vi "Octal Channel Engine.vi"(0 "Notifier Name":string, 11 "AOTF Index":string[](array[string])) -> ()   [LabVIEW 2016]
uses:
  Octal Channel Type Defs/Octal Channel AOTF Config.ctl
  AOTF Controls/AOTF Notifier Element.ctl
  AOTF Controls/AOTF Actions.ctl
  Program Files/Crystal Technology/Developer/AotfLibrary/Dll/AotfLibrary.dll
panel:
  in  "Wavelength (nm)":u16(ring) items=["642", "560", "542"]
  in  "Line On/Off":bool
  out "Controller Response":string
  in  "Blank All":bool=TRUE
  in  "Quit":bool
  in  "Power (%)":dbl
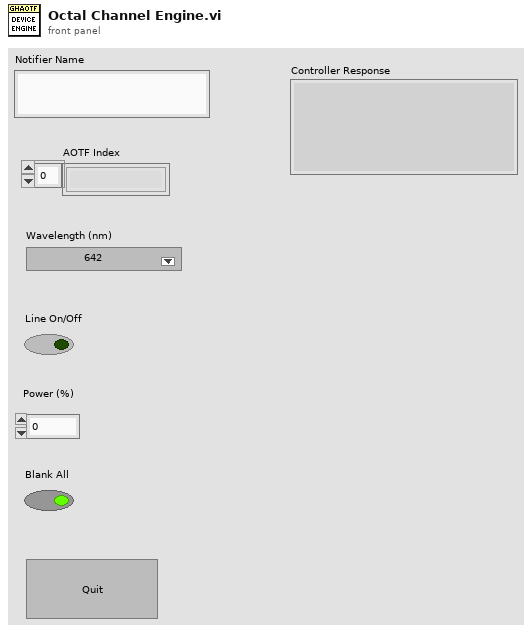
[diagram p1: front panel]
types:
  T1 = typedef "AOTF Notifier Element.ctl" = cluster{"AOTF Action":T2, "Laser Line":string, "Power (%)":dbl, "Beam Blank On/Off":bool, "Line On/Off":bool, "Error":errorcluster, "Wavelengths (nm)":string[]}
  T2 = typedef "AOTF Actions.ctl" = enum16{"Error Check", "Blank", "Line On/Off", "Set Power", "Status", "Quit"}
  T3 = typedef "Octal Channel AOTF Config.ctl" = cluster{"Wavelength (nm)":u16[], "Channel Number":u8[], "Frequency (MHz)":dbl[], "Max Power":dbl[]}
  T4 = enum32{"Invalid", "Standard", "Closed", "Hidden", "Minimized", "Maximized"}
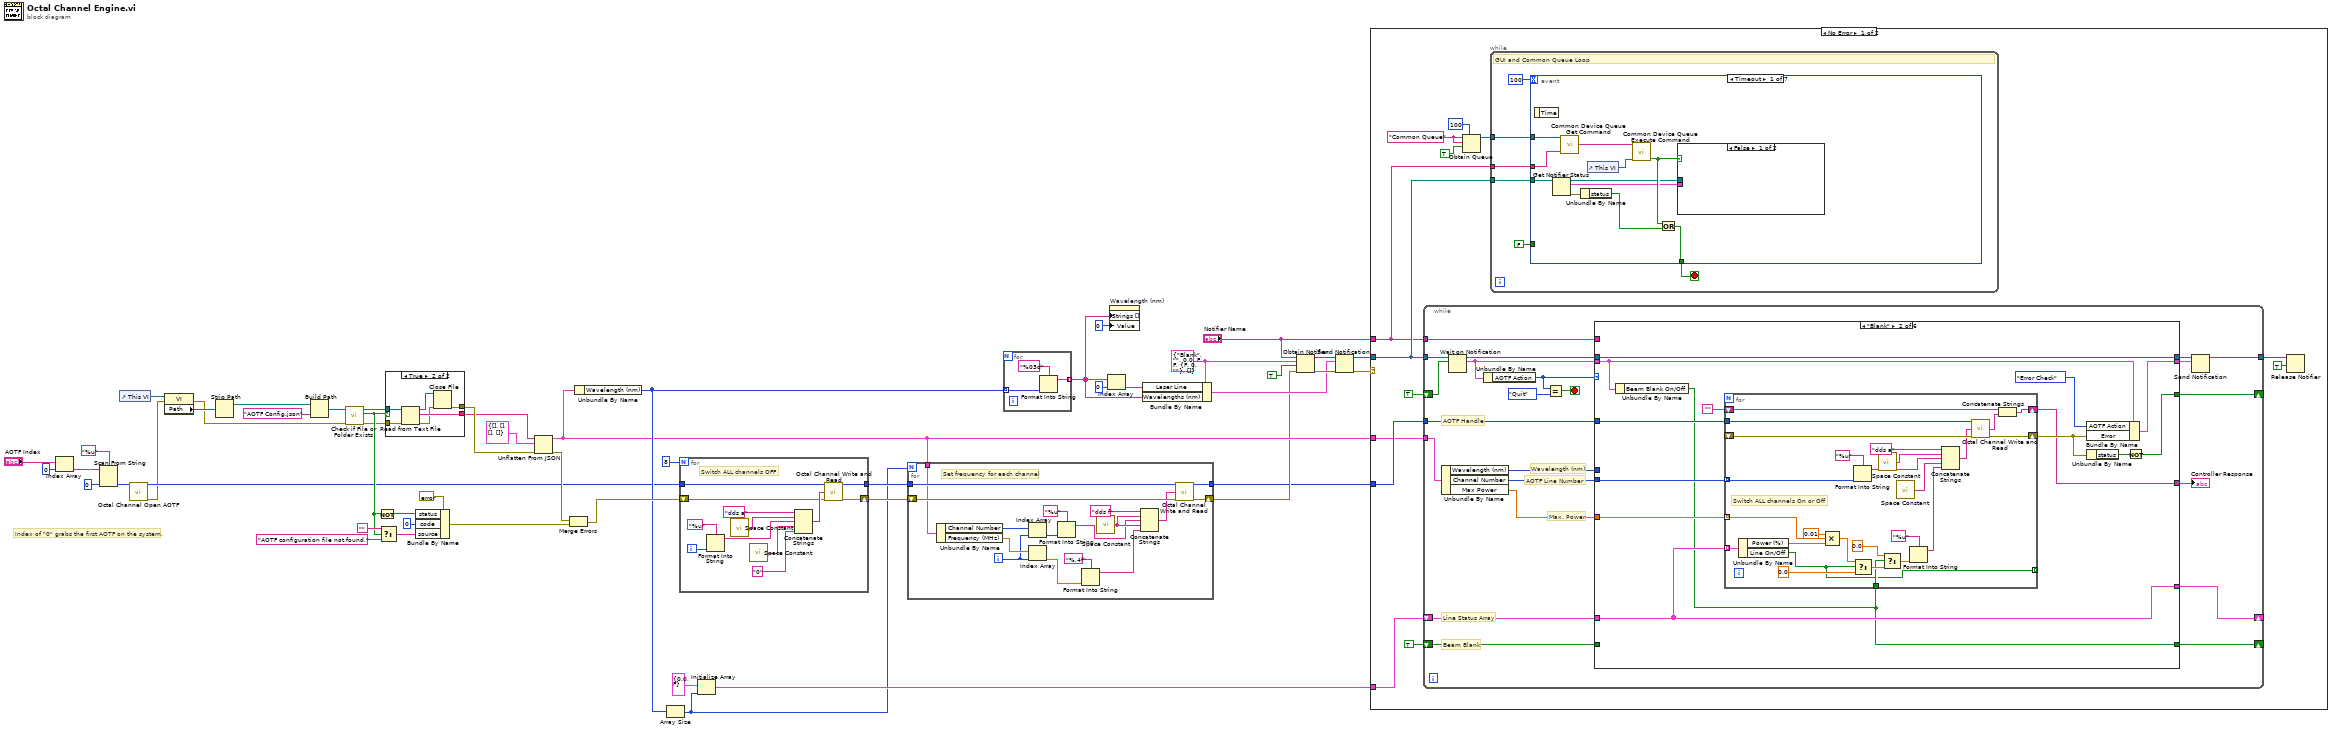
[diagram p0: block diagram]
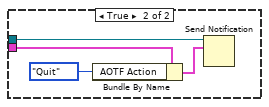
[diagram p2: hidden frame]
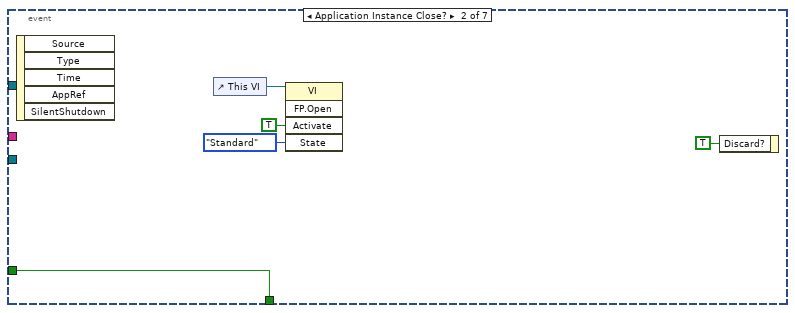
[diagram p3: hidden frame]
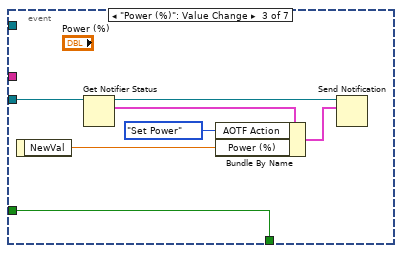
[diagram p4: hidden frame]
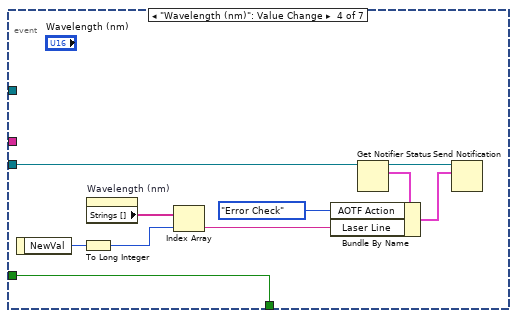
[diagram p5: hidden frame]
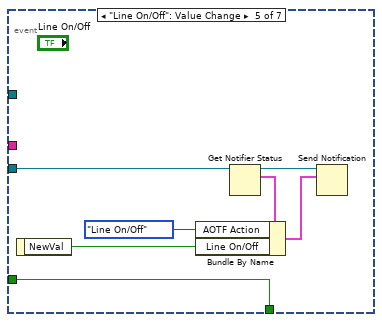
[diagram p6: hidden frame]
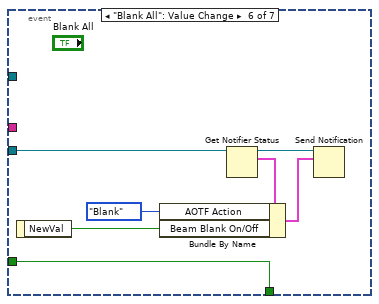
[diagram p7: hidden frame]
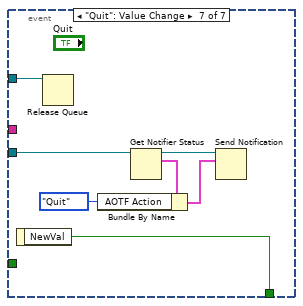
[diagram p8: hidden frame]
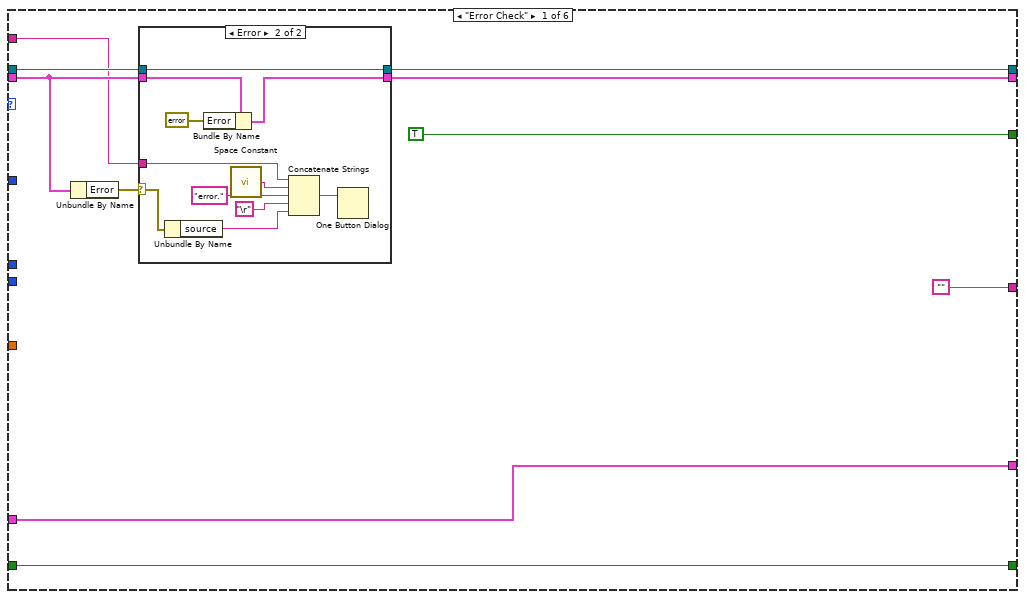
[diagram p9: hidden frame]
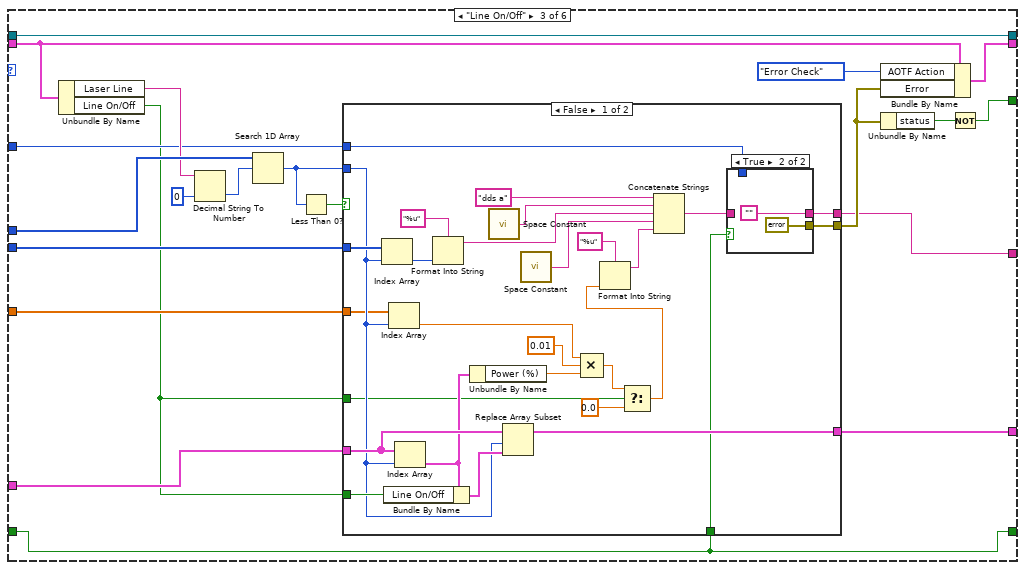
[diagram p11: hidden frame]
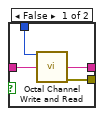
[diagram p12: hidden frame]
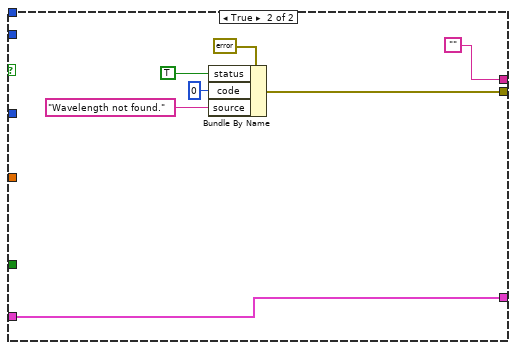
[diagram p13: hidden frame]
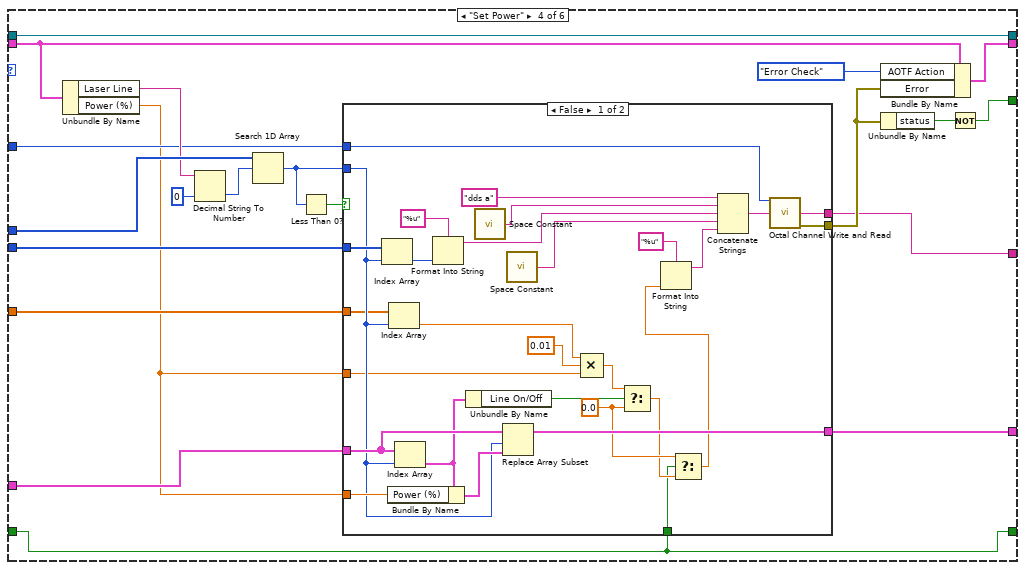
[diagram p14: hidden frame]
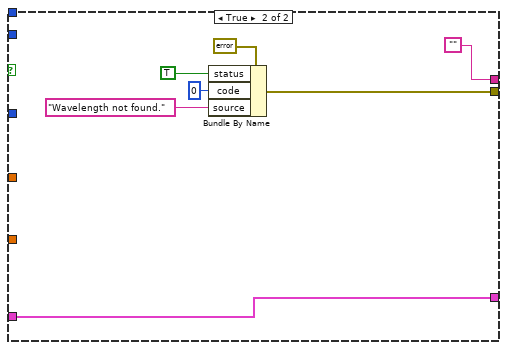
[diagram p15: hidden frame]
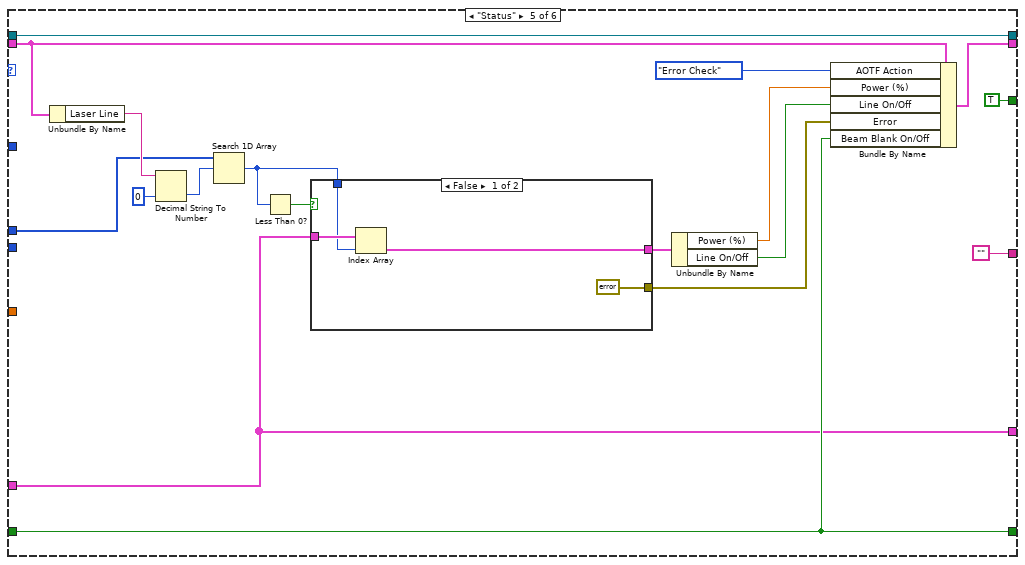
[diagram p16: hidden frame]
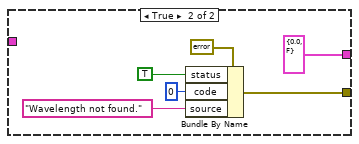
[diagram p17: hidden frame]
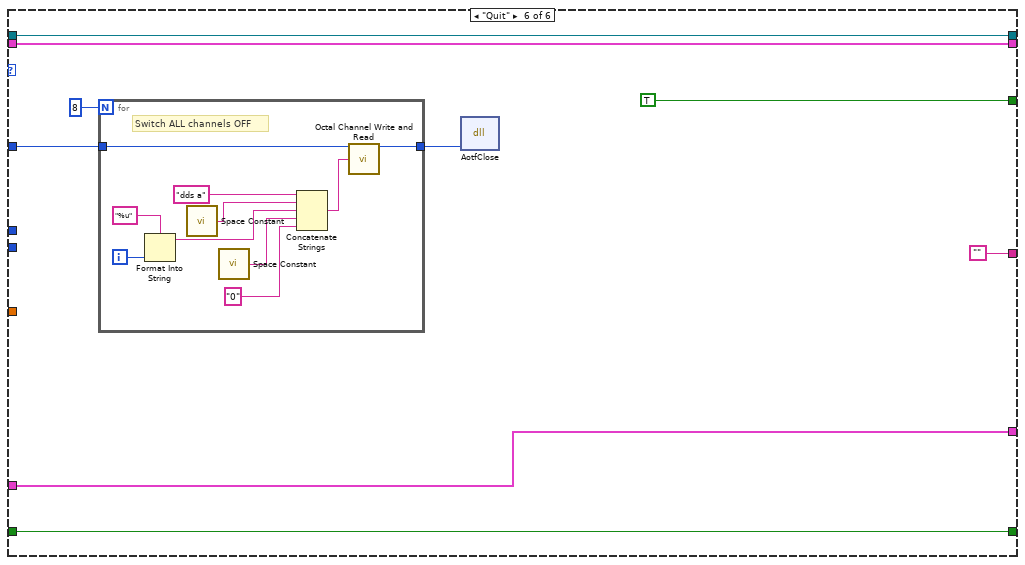
[diagram p18: hidden frame]
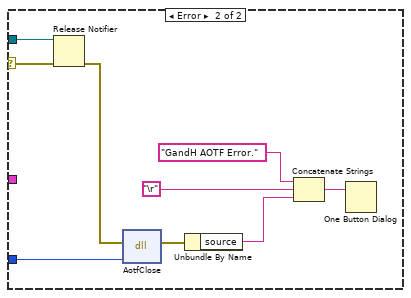
[diagram p19: hidden frame]
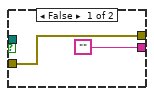
[diagram p20: hidden frame]
diagram:
  w17 = T1 {"AOTF Action"=enum."Blank", "Laser Line"="", "Power (%)"=0.0, "Beam Blank On/Off"=FALSE, "Line On/Off"=FALSE, "Error"={"status"=FALSE, "code"=0, "source"=""}, "Wavelengths (nm)"=[]} ("AOTFQueueCtrl")
  # "Index of \"0\" grabs the first AOTF on the system."
  n1 = Index Array(array="AOTF Index", index=0) -> (element=w4:string)
  n2 = Scan From String(format string="%u", input string=w4, default 1=0 ("AOTF Index")) -> (output 1=w1:i32)  [unwired: 2 in, 3 out]
  n3 = control-ref of="This VI"() -> (w51:refnum<vi>)
  n4 = call "Octal Channel Open AOTF.vi"("AOTF Index"=w1) -> ("AOTF Handle"=w15:u64, "Error Out"=w14:errorcluster)  [unwired: 13 in]
  n5 = property class="VI"(reference=w51, error in=w14) -> (error out=w38:errorcluster, "Path"=w50:path)  [unwired: 1 out]
  n6 = Strip Path(path=w50) -> (stripped path=w49:path)  [unwired: 1 out]
  n7 = Build Path(base path=w49, name or relative path="AOTF Config.json") -> (appended path=w47:path)
  n8 = call <vilib>:"Check if File or Folder Exists.vi"("error in (no error)"=w38, "path"=w47) -> ("error out"=w37:errorcluster, "file or folder exists?"=w40:bool, "dup path"=w39:path)  [unwired: 7 in]
  n9 = Not(x=w40) -> (.not. x?=w45:bool)
  n10 = Select(t="", s=w40, f="AOTF configuration file not found." ("source")) -> (s? t:f=w41:string)
  n11 = case shown="True" w40 {
    tunnel: w39 -> [_ w59]
    tunnel: ["" w58] -> w33
    tunnel: w37 -> [w52 w56]
    tunnel: [w52 w54] -> w36
    frame False {
    }
    frame True {
      n12 = Read from Text File(file (use dialog)=w59, error in=w56) -> (refnum out=w57:refnum<file>, text=w58:string, error out=w55:errorcluster)  [unwired: 2 in, 1 out]
      n13 = Close File(refnum=w57, error in=w55) -> (error out=w54:errorcluster)  [unwired: 1 out]
    }
  }
  n14 = Bundle By Name(cluster=errorcluster {"status"=FALSE, "code"=0, "source"=""} ("Error"), "status"=w45, "code"=0, "source"=w41) -> (w34:errorcluster)
  n15 = Unflatten From JSON(JSON string=w33, type and defaults=T3 {"Wavelength (nm)"=[], "Channel Number"=[], "Frequency (MHz)"=[], "Max Power"=[]} ("AOTF Config"), error in (no error)=w36) -> (value=w9:T3, error out=w35:errorcluster)  [unwired: 4 in]
  n16 = Merge Errors(w35, w34) -> (w29:errorcluster)
  n17 = Unbundle By Name(w9) -> ("Wavelength (nm)"=w28:u16[])
  n18 = Array Size(array=w28) -> (size(s)=w10:i32)
  n19 = for {
    N: 8 -> [_]
    shift-right: [w63] -> w12
    shift-left: w29 -> [w62]
    tunnel: w15 -> [w61]
    tunnel: [w60] -> w11
    i -> [w64]
    # "Switch ALL channels OFF"
    n20 = Format Into String(format string="%u", w64) -> (resulting string=w71:string)  [unwired: 2 in, 1 out]
    n21 = call <vilib>:"Space Constant.vi"() -> ("String"=w66:string)
    n22 = call <vilib>:"Space Constant.vi"() -> ("String"=w67:string)
    n23 = Concatenate Strings("dds a", w66, w71, w67, "0") -> (w69:string)
    n24 = call "Octal Channel Write and Read.vi"("hAotfController"=w61, "Command"=w69, "Error In"=w62) -> ("hAotfController (Dup)"=w60:u64, "Error Out"=w63:errorcluster)  [unwired: 10 in, 1 out]
  }
  n25 = Initialize Array(cluster{"Power (%)":dbl, "Line On/Off":bool} {"Power (%)"=0.0, "Line On/Off"=FALSE} ("Line Staus Cluster"), w10) -> (w30:cluster{"Power (%)":dbl, "Line On/Off":bool}[])
  n26 = for {
    N: w10 -> [_]
    shift-right: [w80] -> w8
    shift-left: w12 -> [w87]
    tunnel: w11 -> [w88]
    tunnel: w9 -> [w86]
    tunnel: [w72] -> w7
    i -> [w83]
    # "Set frequency for each channel"
    n27 = Unbundle By Name(w86) -> ("Channel Number"=w85:u8[], "Frequency (MHz)"=w84:dbl[])
    n28 = Index Array(array=w85, index=w83) -> (element=w77:u8)
    n29 = Index Array(array=w84, index=w83) -> (element=w74:dbl)
    n30 = Format Into String(format string="%u", w77) -> (resulting string=w76:string)  [unwired: 2 in, 1 out]
    n31 = Format Into String(format string="%.4f", w74) -> (resulting string=w73:string)  [unwired: 2 in, 1 out]
    n32 = call <vilib>:"Space Constant.vi"() -> ("String"=w81:string)
    n33 = Concatenate Strings("dds f", w81, w76, w81, w73) -> (w79:string)
    n34 = call "Octal Channel Write and Read.vi"("hAotfController"=w88, "Command"=w79, "Error In"=w87) -> ("hAotfController (Dup)"=w72:u64, "Error Out"=w80:errorcluster)  [unwired: 10 in, 1 out]
  }
  n35 = for {
    tunnel: w28 -> [w91] mode=indexing
    tunnel: [w90] -> w27 mode=indexing
    n36 = Format Into String(format string="%03d", w91) -> (resulting string=w90:string)  [unwired: 2 in, 1 out]
  }
  n37 = Index Array(array=w27, index=0) -> (element=w25:string)
  n38 = property on="Wavelength (nm)" class="Ring (strict)"("Strings []"=w27, "Value"=u16 0 ("index")) -> ()  [unwired: 2 in, 2 out]
  n39 = Bundle By Name(cluster=w17, "Laser Line"=w25, "Wavelengths (nm)"=w27) -> (w16:T1)
  n40 = Obtain Notifier(name (unnamed)="Notifier Name", notification data type=w17, create if not found? (T)=TRUE, error in (no error)=w8) -> (notifier out=w21:refnum<notifier>, error out=w20:errorcluster)  [unwired: 1 out]
  n41 = Send Notification(notification=w16, notifier=w21, error in (no error)=w20) -> (notifier out=w19:refnum<notifier>, error out=w18:errorcluster)
  n42 = case shown="No Error" w18 {
    selector: w18 -> [_ w427]
    tunnel: w19 -> [w100 w428]
    tunnel: "Notifier Name" -> [w96 _]
    tunnel: w7 -> [w95 w420]
    tunnel: w30 -> [w94 _]
    tunnel: w9 -> [w92 _]
    frame No Error {
      w104 = "Common Queue" ("Unique Notifier Name")
      n43 = while {
        tunnel: w100 -> [w190]
        shift-right: [w181] -> _
        shift-left: TRUE ("ignore previous (F)") -> [w189]
        tunnel: [w180] -> w98
        tunnel: w96 -> [w179]
        tunnel: w95 -> [w178]
        shift-right: [w173] -> _
        shift-left: w94 -> [w176]
        shift-right: [w174] -> _
        shift-left: TRUE -> [w175]
        tunnel: w92 -> [w172]
        stop <- w184 stop-if-true
        # "Wavelength (nm)"
        # "AOTF Line Number"
        # "Line Status Array"
        # "Beam Blank"
        # "AOTF Handle"
        # "Max. Power"
        n44 = Unbundle By Name(w172) -> ("Wavelength (nm)"=w171:u16[], "Channel Number"=w170:u8[], "Max Power"=w169:dbl[])
        n45 = Wait on Notification(notifier=w190, ignore previous (F)=w189) -> (notifier out=w188:refnum<notifier>, notification=w187:T1)  [unwired: 2 in, 2 out]
        n46 = Unbundle By Name(w187) -> ("AOTF Action"=w186:T2)
        n47 = Equal?(x=w186, y=AOTF_Actions."Quit") -> (x = y?=w184:bool)
        n48 = case shown="\"Blank\"" w186 {
          tunnel: w188 -> [w200 w227 w270 w332 w389 w409]
          tunnel: w187 -> [w198 w226 w272 w334 w384 w408]
          tunnel: [w196 w227 w270 w332 w389 w409] -> w183
          tunnel: [w195 w225 w271 w333 w380 w408] -> w182
          tunnel: [TRUE w222 w262 w324 TRUE TRUE] -> w181
          tunnel: w179 -> [w197 _ _ _ _ _]
          tunnel: w171 -> [_ _ w267 w329 w385 _]
          tunnel: w170 -> [_ w220 w264 w326 _ _]
          tunnel: w169 -> [_ w218 w257 w319 _ _]
          tunnel: w178 -> [_ w221 w258 w320 _ w402]
          tunnel: ["" w214 w255 w317 "" ""] -> w177
          tunnel: w176 -> [w192 w217 w261 w323 w373 w405]
          tunnel: w175 -> [w191 _ w254 w316 w374 w404]
          tunnel: [w191 w215 w254 w316 w374 w404] -> w174
          tunnel: [w192 w217 w260 w322 w373 w405] -> w173
          frame "Error Check" {
            n49 = Unbundle By Name(w198) -> ("Error"=w199:errorcluster)
            n50 = case shown="Error" w199 {
              selector: w199 -> [_ w206]
              tunnel: w198 -> [w201 w210]
              tunnel: [w202 w208] -> w196
              tunnel: w200 -> [w202 w208]
              tunnel: w197 -> [_ w205]
              tunnel: [w201 w207] -> w195
              frame No Error {
              }
              frame Error {
                n51 = Unbundle By Name(w206) -> ("source"=w204:string)
                n52 = Bundle By Name(cluster=w210, "Error"=errorcluster {"status"=FALSE, "code"=0, "source"=""}) -> (w207:T1)
                n53 = call <vilib>:"Space Constant.vi"() -> ("String"=w213:string)
                n54 = Concatenate Strings(w205, w213, "error." ("string"), "\r", w204) -> (w211:string)
                n55 = One Button Dialog(message=w211) -> ()  [unwired: 1 in, 1 out]
              }
            }
          }
          frame "Blank" {
            n56 = Unbundle By Name(w226) -> ("Beam Blank On/Off"=w215:bool)
            n57 = for {
              shift-right: [w248] -> w219
              shift-left: _ -> [w247]
              tunnel: w221 -> [w246]
              tunnel: w217 -> [w244] mode=indexing
              tunnel: w220 -> [w245] mode=indexing
              tunnel: w218 -> [w242] mode=indexing
              tunnel: w215 -> [w238]
              shift-right: [w233] -> w214
              shift-left: "" -> [w234]
              tunnel: [w229] -> _ mode=indexing
              # "Switch ALL channels On or Off"
              n58 = Unbundle By Name(w244) -> ("Power (%)"=w228:dbl, "Line On/Off"=w229:bool)
              n59 = Compound Arithmetic op=MULTIPLY(0.01 ("value"), w242, w228) -> (w241:dbl)
              n60 = Format Into String(format string="%u", w245) -> (resulting string=w253:string)  [unwired: 2 in, 1 out]
              n61 = Select(t=w241, s=w229, f=0.0) -> (s? t:f=w239:dbl)
              n62 = call <vilib>:"Space Constant.vi"() -> ("String"=w250:string)
              n63 = Select(t=0.0, s=w238, f=w239) -> (s? t:f=w236:dbl)
              n64 = call <vilib>:"Space Constant.vi"() -> ("String"=w251:string)
              n65 = Format Into String(format string="%u", w236) -> (resulting string=w235:string)  [unwired: 2 in, 1 out]
              n66 = Concatenate Strings("dds a", w250, w253, w251, w235) -> (w230:string)
              n67 = call "Octal Channel Write and Read.vi"("hAotfController"=w246, "Command"=w230, "Error In"=w247) -> ("Response"=w232:string, "Error Out"=w248:errorcluster)  [unwired: 10 in, 1 out]
              n68 = Concatenate Strings(w234, w232) -> (w233:string)
            }
            n69 = Bundle By Name(cluster=w226, "AOTF Action"=AOTF_Actions."Error Check", "Error"=w219) -> (w225:T1)
            n70 = Unbundle By Name(w219) -> ("status"=w223:bool)
            n71 = Not(x=w223) -> (.not. x?=w222:bool)
          }
          frame "Line On/Off" {
            n72 = Unbundle By Name(w272) -> ("Laser Line"=w266:string, "Line On/Off"=w256:bool)
            n73 = Decimal String To Number(string=w266, default (0L)=u16 0 ("default (0 I32)")) -> (number=w269:u16)  [unwired: 1 in, 1 out]
            n74 = Search 1D Array(1D array=w267, element=w269) -> (index of element=w259:i32)  [unwired: 1 in]
            n75 = Less Than 0?(x=w259) -> (x < 0?=w265:bool)
            n76 = case shown="False" w265 {
              tunnel: w264 -> [w302 _]
              tunnel: [w297 w311] -> w263
              tunnel: [w278 ""] -> w255
              tunnel: w261 -> [w301 w309]
              tunnel: [w300 w309] -> w260
              tunnel: w256 -> [w298 _]
              tunnel: w259 -> [w288 _]
              tunnel: w258 -> [w289 _]
              tunnel: w257 -> [w287 _]
              tunnel: w256 -> [w281 _]
              tunnel: w254 -> [w275 _]
              frame False {
                n77 = Index Array(array=w302, index=w288) -> (element=w291:u8)
                n78 = Index Array(array=w287, index=w288) -> (element=w282:dbl)
                n79 = Index Array(array=w301, index=w288) -> (element=w285:cluster{"Power (%)":dbl, "Line On/Off":bool})
                n80 = Bundle By Name(cluster=w285, "Line On/Off"=w298) -> (w299:cluster{"Power (%)":dbl, "Line On/Off":bool})
                n81 = Format Into String(format string="%u", w291) -> (resulting string=w292:string)  [unwired: 2 in, 1 out]
                n82 = Unbundle By Name(w285) -> ("Power (%)"=w284:dbl)
                n83 = call <vilib>:"Space Constant.vi"() -> ("String"=w295:string)
                n84 = Replace Array Subset(array=w301, new element=w299, index=w288) -> (w300:cluster{"Power (%)":dbl, "Line On/Off":bool}[])
                n85 = call <vilib>:"Space Constant.vi"() -> ("String"=w294:string)
                n86 = Compound Arithmetic op=MULTIPLY(w282, 0.01 ("value"), w284) -> (w286:dbl)
                n87 = Select(t=w286, s=w281, f=0.0) -> (s? t:f=w276:dbl)
                n88 = Format Into String(format string="%u", w276) -> (resulting string=w279:string)  [unwired: 2 in, 1 out]
                n89 = Concatenate Strings("dds a", w295, w292, w294, w279) -> (w290:string)
                n90 = case shown="True" w275 {
                  tunnel: [w306 errorcluster {"status"=FALSE, "code"=0, "source"=""} ("Error Out")] -> w297
                  tunnel: w290 -> [w305 _]
                  tunnel: w289 -> [w304 _]
                  tunnel: [w303 ""] -> w278
                  frame False {
                    n91 = call "Octal Channel Write and Read.vi"("hAotfController"=w304, "Command"=w305) -> ("Response"=w303:string, "Error Out"=w306:errorcluster)  [unwired: 11 in, 1 out]
                  }
                  frame True {
                  }
                }
              }
              frame True {
                n92 = Bundle By Name(cluster=errorcluster {"status"=FALSE, "code"=0, "source"=""} ("error out"), "status"=TRUE, "code"=0, "source"="Wavelength not found.") -> (w311:errorcluster)
              }
            }
            n93 = Bundle By Name(cluster=w272, "AOTF Action"=AOTF_Actions."Error Check", "Error"=w263) -> (w271:T1)
            n94 = Unbundle By Name(w263) -> ("status"=w273:bool)
            n95 = Not(x=w273) -> (.not. x?=w262:bool)
          }
          frame "Set Power" {
            n96 = Unbundle By Name(w334) -> ("Laser Line"=w328:string, "Power (%)"=w318:dbl)
            n97 = Decimal String To Number(string=w328, default (0L)=u16 0 ("default (0 I32)")) -> (number=w331:u16)  [unwired: 1 in, 1 out]
            n98 = Search 1D Array(1D array=w329, element=w331) -> (index of element=w321:i32)  [unwired: 1 in]
            n99 = Less Than 0?(x=w321) -> (x < 0?=w327:bool)
            n100 = case shown="False" w327 {
              tunnel: w326 -> [w365 _]
              tunnel: [w360 w368] -> w325
              tunnel: [w343 ""] -> w317
              tunnel: w323 -> [w364 w366]
              tunnel: [w363 w366] -> w322
              tunnel: w318 -> [w361 _]
              tunnel: w321 -> [w351 _]
              tunnel: w320 -> [w352 _]
              tunnel: w319 -> [w350 _]
              tunnel: w318 -> [w341 _]
              tunnel: w316 -> [w338 _]
              frame False {
                w340 = 0.0
                n101 = Index Array(array=w365, index=w351) -> (element=w354:u8)
                n102 = Index Array(array=w350, index=w351) -> (element=w346:dbl)
                n103 = Index Array(array=w364, index=w351) -> (element=w348:cluster{"Power (%)":dbl, "Line On/Off":bool})
                n104 = Bundle By Name(cluster=w348, "Power (%)"=w361) -> (w362:cluster{"Power (%)":dbl, "Line On/Off":bool})
                n105 = Format Into String(format string="%u", w354) -> (resulting string=w355:string)  [unwired: 2 in, 1 out]
                n106 = Unbundle By Name(w348) -> ("Line On/Off"=w342:bool)
                n107 = call <vilib>:"Space Constant.vi"() -> ("String"=w358:string)
                n108 = Replace Array Subset(array=w364, new element=w362, index=w351) -> (w363:cluster{"Power (%)":dbl, "Line On/Off":bool}[])
                n109 = call <vilib>:"Space Constant.vi"() -> ("String"=w357:string)
                n110 = Compound Arithmetic op=MULTIPLY(w346, 0.01 ("value"), w341) -> (w349:dbl)
                n111 = Select(t=w349, s=w342, f=w340) -> (s? t:f=w339:dbl)
                n112 = Select(t=w340, s=w338, f=w339) -> (s? t:f=w337:dbl)
                n113 = Format Into String(format string="%u", w337) -> (resulting string=w344:string)  [unwired: 2 in, 1 out]
                n114 = Concatenate Strings("dds a", w358, w355, w357, w344) -> (w353:string)
                n115 = call "Octal Channel Write and Read.vi"("hAotfController"=w352, "Command"=w353) -> ("Response"=w343:string, "Error Out"=w360:errorcluster)  [unwired: 11 in, 1 out]
              }
              frame True {
                n116 = Bundle By Name(cluster=errorcluster {"status"=FALSE, "code"=0, "source"=""} ("error out"), "status"=TRUE, "code"=0, "source"="Wavelength not found.") -> (w368:errorcluster)
              }
            }
            n117 = Bundle By Name(cluster=w334, "AOTF Action"=AOTF_Actions."Error Check", "Error"=w325) -> (w333:T1)
            n118 = Unbundle By Name(w325) -> ("status"=w335:bool)
            n119 = Not(x=w335) -> (.not. x?=w324:bool)
          }
          frame "Status" {
            n120 = Unbundle By Name(w384) -> ("Laser Line"=w386:string)
            n121 = Decimal String To Number(string=w386, default (0L)=u16 0 ("default (0 I32)")) -> (number=w387:u16)  [unwired: 1 in, 1 out]
            n122 = Search 1D Array(1D array=w385, element=w387) -> (index of element=w382:i32)  [unwired: 1 in]
            n123 = Less Than 0?(x=w382) -> (x < 0?=w383:bool)
            n124 = case shown="False" w383 {
              tunnel: w373 -> [w394 _]
              tunnel: [errorcluster {"status"=FALSE, "code"=0, "source"=""} ("error out") w396] -> w378
              tunnel: w382 -> [w393 _]
              tunnel: [w392 cluster{"Power (%)":dbl, "Line On/Off":bool} {"Power (%)"=0.0, "Line On/Off"=FALSE} ("Line Staus Cluster")] -> w377
              frame False {
                n125 = Index Array(array=w394, index=w393) -> (element=w392:cluster{"Power (%)":dbl, "Line On/Off":bool})
              }
              frame True {
                n126 = Bundle By Name(cluster=errorcluster {"status"=FALSE, "code"=0, "source"=""} ("error out"), "status"=TRUE, "code"=0, "source"="Wavelength not found.") -> (w396:errorcluster)
              }
            }
            n127 = Unbundle By Name(w377) -> ("Power (%)"=w376:dbl, "Line On/Off"=w375:bool)
            n128 = Bundle By Name(cluster=w384, "AOTF Action"=AOTF_Actions."Error Check", "Power (%)"=w376, "Line On/Off"=w375, "Error"=w378, "Beam Blank On/Off"=w374) -> (w380:T1)
          }
          frame "Quit" {
            n129 = for {
              N: 8 -> [_]
              tunnel: w402 -> [w411]
              tunnel: [w410] -> w401
              i -> [w412]
              # "Switch ALL channels OFF"
              n130 = Format Into String(format string="%u", w412) -> (resulting string=w419:string)  [unwired: 2 in, 1 out]
              n131 = call <vilib>:"Space Constant.vi"() -> ("String"=w414:string)
              n132 = call <vilib>:"Space Constant.vi"() -> ("String"=w415:string)
              n133 = Concatenate Strings("dds a", w414, w419, w415, "0") -> (w417:string)
              n134 = call "Octal Channel Write and Read.vi"("hAotfController"=w411, "Command"=w417) -> ("hAotfController (Dup)"=w410:u64)  [unwired: 11 in, 2 out]
            }
            n135 = dll-call lib="C:/Program Files/Crystal Technology/Developer/AotfLibrary/Dll/AotfLibrary.dll" fn="AotfClose"("hAotfContoller"=w401) -> ()  [unwired: 5 in, 2 out]
          }
        }
        "Controller Response" <- w177
        n136 = Send Notification(notification=w182, notifier=w183) -> (notifier out=w180:refnum<notifier>)  [unwired: 1 in, 1 out]
      }
      n137 = Obtain Queue(max queue size (-1, unlimited)=100, name (unnamed)=w104, element data type=w104, create if not found? (T)=TRUE) -> (queue out=w101:refnum<queue>)  [unwired: 1 in, 2 out]
      n138 = while {
        tunnel: w101 -> [w109]
        tunnel: w96 -> [w107]
        tunnel: w100 -> [w108]
        stop <- w106 stop-if-true
        # "GUI and Common Queue Loop"
        n139 = event shown="[0] Timeout" {
          selector: _ -> [_ _ _ _ _ _ _]
          dyn-events: _ -> [_ _ _ _ _ _ _]
          timeout: 100 -> [_ _ _ _ _ _ _]
          tunnel: w109 -> [w116 _ _ _ _ _ w168]
          tunnel: w108 -> [w112 _ w133 w144 w150 w160 w167]
          tunnel: w107 -> [w115 _ _ _ _ _ _]
          tunnel: [w114 w130 w137 w147 w154 w161 w165] -> w106
          tunnel: FALSE -> [_ w130 w137 w147 w154 w161 _]
          event Timeout {
            n140 = event-data() -> ()  [unwired: 1 in, 1 out]
            n141 = Get Notifier Status(notifier=w112) -> (notifier out=w111:refnum<notifier>, current notification=w113:T1, error out=w121:errorcluster)  [unwired: 1 in, 2 out]
            n142 = call "Common Device Queue Get Command.vi"("Common Queue"=w116, "Notifier Name"=w115) -> ("Command"=w120:string)  [unwired: 12 in, 1 out]
            n143 = Unbundle By Name(w121) -> ("status"=w118:bool)
            n144 = control-ref of="This VI"() -> (w119:refnum<vi>)
            n145 = call "Common Device Queue Execute Command.vi"("Common Command"=w120, "VI Refnum"=w119) -> ("Quit?"=w117:bool)  [unwired: 12 in, 1 out]
            n146 = Or(x=w117, y=w118) -> (x .or. y?=w114:bool)
            n147 = case shown="False" w117 {
              tunnel: w111 -> [_ w125]
              tunnel: w113 -> [_ w124]
              frame False {
              }
              frame True {
                n148 = Bundle By Name(cluster=w124, "AOTF Action"=AOTF_Actions."Quit") -> (w123:T1)
                n149 = Send Notification(notification=w123, notifier=w125) -> ()  [unwired: 1 in, 2 out]
              }
            }
          }
          event Application Instance Close? {
            n150 = event-data() -> ()  [unwired: 1 in, 5 out]
            n151 = control-ref of="This VI"() -> (w127:refnum<vi>)
            n152 = invoke class="VI" method="FP.Open"(reference=w127, "Activate"=TRUE ("Activate?"), "State"=T4."Standard") -> ()  [unwired: 2 in, 5 out]
            n153 = event-data("Discard?"=TRUE) -> ()  [unwired: 1 in, 1 out]
          }
          event "Power (%)": Value Change {
            n154 = event-data() -> ("NewVal"=w135:dbl)  [unwired: 1 in]
            n155 = Get Notifier Status(notifier=w133) -> (notifier out=w131:refnum<notifier>, current notification=w132:T1)  [unwired: 1 in, 3 out]
            n156 = Bundle By Name(cluster=w132, "AOTF Action"=AOTF_Actions."Set Power", "Power (%)"=w135) -> (w134:T1)
            n157 = Send Notification(notification=w134, notifier=w131) -> ()  [unwired: 1 in, 2 out]
          }
          event "Wavelength (nm)": Value Change {
            n158 = event-data() -> ("NewVal"=w140:u16)  [unwired: 1 in]
            n159 = To Long Integer(number=w140) -> (32bit integer=w139:i32)
            n160 = property on="Wavelength (nm)" class="Ring (strict)"() -> ("Strings []"=w141:string[])  [unwired: 2 in, 2 out]
            n161 = Index Array(array=w141, index=w139) -> (element=w138:string)
            n162 = Get Notifier Status(notifier=w144) -> (notifier out=w142:refnum<notifier>, current notification=w143:T1)  [unwired: 1 in, 3 out]
            n163 = Bundle By Name(cluster=w143, "AOTF Action"=AOTF_Actions."Error Check", "Laser Line"=w138) -> (w145:T1)
            n164 = Send Notification(notification=w145, notifier=w142) -> ()  [unwired: 1 in, 2 out]
          }
          event "Line On/Off": Value Change {
            n165 = event-data() -> ("NewVal"=w149:bool)  [unwired: 1 in]
            n166 = Get Notifier Status(notifier=w150) -> (notifier out=w153:refnum<notifier>, current notification=w152:T1)  [unwired: 1 in, 3 out]
            n167 = Bundle By Name(cluster=w152, "AOTF Action"=AOTF_Actions."Line On/Off", "Line On/Off"=w149) -> (w148:T1)
            n168 = Send Notification(notification=w148, notifier=w153) -> ()  [unwired: 1 in, 2 out]
          }
          event "Blank All": Value Change {
            n169 = event-data() -> ("NewVal"=w156:bool)  [unwired: 1 in]
            n170 = Get Notifier Status(notifier=w160) -> (notifier out=w159:refnum<notifier>, current notification=w158:T1)  [unwired: 1 in, 3 out]
            n171 = Bundle By Name(cluster=w158, "AOTF Action"=AOTF_Actions."Blank", "Beam Blank On/Off"=w156) -> (w155:T1)
            n172 = Send Notification(notification=w155, notifier=w159) -> ()  [unwired: 1 in, 2 out]
          }
          event "Quit": Value Change {
            n173 = event-data() -> ("NewVal"=w165:bool)  [unwired: 1 in]
            n174 = Release Queue(queue=w168) -> ()  [unwired: 2 in, 3 out]
            n175 = Get Notifier Status(notifier=w167) -> (notifier out=w166:refnum<notifier>, current notification=w164:T1)  [unwired: 1 in, 3 out]
            n176 = Bundle By Name(cluster=w164, "AOTF Action"=AOTF_Actions."Quit") -> (w162:T1)
            n177 = Send Notification(notification=w162, notifier=w166) -> ()  [unwired: 1 in, 2 out]
          }
        }
      }
      n178 = Release Notifier(notifier=w98, force destroy? (F)=TRUE) -> ()  [unwired: 1 in, 3 out]
    }
    frame Error {
      n179 = Release Notifier(notifier=w428, error in (no error)=w427) -> (error out=w422:errorcluster)  [unwired: 1 in, 2 out]
      n180 = dll-call lib="C:/Program Files/Crystal Technology/Developer/AotfLibrary/Dll/AotfLibrary.dll" fn="AotfClose"(error in=w422, "hAotfContoller"=w420) -> (error out=w421:errorcluster)  [unwired: 4 in, 1 out]
      n181 = Unbundle By Name(w421) -> ("source"=w424:string)
      n182 = Concatenate Strings("GandH AOTF Error.", "\r", w424) -> (w423:string)
      n183 = One Button Dialog(message=w423) -> ()  [unwired: 1 in, 1 out]
    }
  }
